vi "Test View No Process Errors Showing and Hiding Panel.vi"(8 "error in (no error)":errorcluster, 11 "UI View Test In":refnum<class "View Test.lvclass">) -> (0 "error out":errorcluster, 3 "UI View Test Out":refnum<class "View Test.lvclass">)   [LabVIEW 2020, in "View Test.lvclass"]
uses:
  View Test.lvclass
  C:/Program Files (x86)/National Instruments/LabVIEW 2020/vi.lib/Astemes/LUnit/Test Case.lvclass
  Mock Error Handler/Mock Error Handler.lvclass
  C:/Git/astemes-triarc-framework/source/Framework/Error Handler Interface/Error Handler Interface.lvclass
  Framework/Process/Process.lvclass/Process.ctl
  Framework/View/View.lvclass/View.ctl
  <vilib>/Astemes/LUnit/Test Case.lvclass/Test Case.ctl
  Framework/Process/Protected/Messaging/Send Message.vi
  Framework/Process/Public/Lifecycle/Get Lifecycle State.vi
  Framework/View/Public/Get View VI Reference.vi
  <vilib>/Utility/error.llb/Clear Errors.vi
  Framework/Broadcast Event Helpers/Execution timer.vi
  Framework/Process/Private/SubVIs/Wait for finish.vi
  Framework/Process/Private/SubVIs/Set Lifecycle State.vi
  <vilib>/Astemes/LUnit/Palette/Pass.vi
  <vilib>/Astemes/LUnit/Palette/Fail.vi
  <vilib>/Astemes/LUnit/Set Assertion Type.vi
  Framework/Process/Private/SubVIs/Handle Debug Data.vi
  Framework/Process/Protected/Messaging/Request Message.vi
  <vilib>/Astemes/LUnit/Add test result.vi
  Framework/Logging/Log Debug.vi
  <vilib>/AdvancedString/1D String Array to Delimited String.vi
  <vilib>/Utility/High Resolution Relative Seconds.vi
  Framework/Process/Private/SubVIs/Enqueue Request Message.vi
  <vilib>/Astemes/LUnit/LUnit Record Assertion Result.vi
  <vilib>/Astemes/LUnit/LUnit Aggregate Assertion Results.vi
  <vilib>/Astemes/LUnit/Method Result/LUnit Merge Status.vi
  <vilib>/Astemes/LUnit/LUnit Concatenate result strings.vi
  Framework/View/View.lvclass
  C:/Git/astemes-triarc-framework/source/Framework/Process/Process.lvclass
  <vilib>/Utility/error.llb/Error Cluster From Error Code.vi
  Framework/Process/Public/Read Name.vi
  Framework/Process/Private/SubVIs/Wait for Response Message.vi
  Framework/Broadcast Event Helpers/Dequeue Broadcast Message.vi
  Framework/Process/Process.lvclass
  View Test.lvclass/View Test.ctl
  <vilib>/Astemes/LUnit/Test Case.lvclass
  C:/Git/astemes-triarc-framework/source/Framework/Base/Base.lvclass
  C:/Git/astemes-triarc-framework/source/Framework/Logging/Logging.lvclass
  C:/Git/astemes-triarc-framework/source/Framework/View/View.lvclass
  Framework/Broadcast Event Helpers/Broadcast Event Helpers.lvlib
  C:/Git/astemes-triarc-framework/source/Framework Test Suite/Process Test/Process Test.lvclass
  C:/Git/astemes-triarc-framework/source/Framework Test Suite/Base Class Test/Base Test.lvclass
  C:/Git/astemes-triarc-framework/source/Framework Test Suite/View Test/View Test.lvclass
  Process Test/Process Test.lvclass
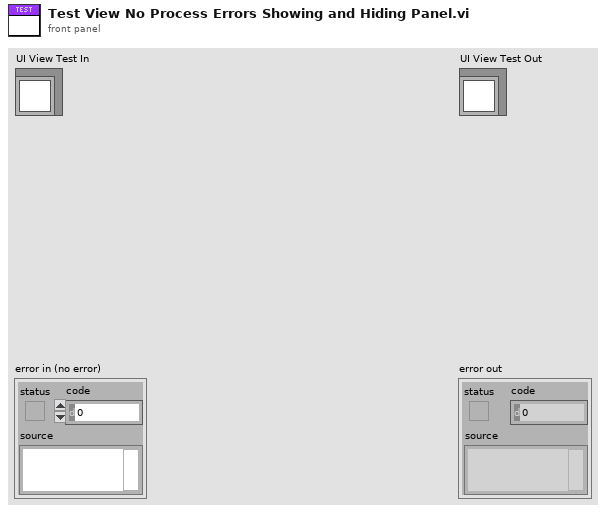
[diagram p1: front panel]
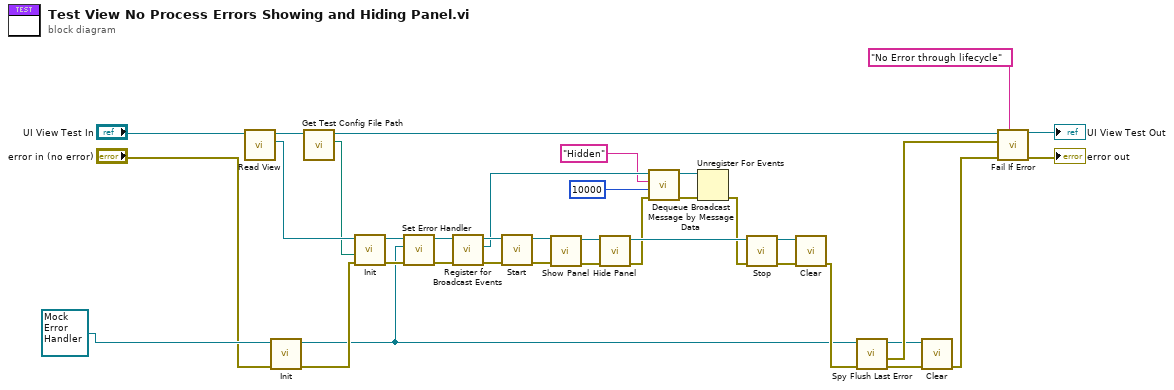
[diagram p0: block diagram]
diagram:
  n1 = call "Read View.vi"("View Test In"="UI View Test In") -> ("View"=w30:refnum<class "View.lvclass">, "View Test Out"=w35:refnum<class "View Test.lvclass">)  [unwired: 8 in, 1 out]
  n2 = call-dynamic "Init.vi"("error in (no error)"="error in (no error)", "Mock Error Handler In"=refnum<class "Mock Error Handler.lvclass"> refnum ("Mock Error Handler.lvclass")) -> ("error out"=w21:errorcluster, "Mock Error Handler Out"=w14:refnum<class "Mock Error Handler.lvclass">)  [unwired: 8 in]
  n3 = call "Get Test Config File Path.vi"("Process Test In"=w35) -> ("Test config path"=w1:path, "Process Test Out"=w2:refnum<class "View Test.lvclass">)  [unwired: 8 in, 1 out]
  n4 = call-dynamic "Init.vi"("error in (no error)"=w21, "Config File Path"=w1, "View In"=w30) -> ("error out"=w24:errorcluster, "View Out"=w32:refnum<class "View.lvclass">)  [unwired: 7 in]
  n5 = call "Set Error Handler.vi"("error in (no error)"=w24, "Error Handler"=w14, "Process In"=w32) -> ("error out"=w23:errorcluster, "Process Out"=w11:refnum<class "View.lvclass">)  [unwired: 7 in]
  n6 = call "Register for Broadcast Events.vi"("error in (no error)"=w23, "Process In"=w11) -> ("error out"=w12:errorcluster, "Event Registration Refnum Out"=w9:refnum<event-registration>, "Process Out"=w10:refnum<class "View.lvclass">)  [unwired: 7 in]
  n7 = call "Start.vi"("error in (no error)"=w12, "Process In"=w10) -> ("error out"=w28:errorcluster, "Process Out"=w29:refnum<class "View.lvclass">)  [unwired: 7 in, 1 out]
  n8 = call "Show Panel.vi"("error in (no error)"=w28, "View In"=w29) -> ("error out"=w16:errorcluster, "View Out"=w17:refnum<class "View.lvclass">)  [unwired: 8 in]
  n9 = call "Hide Panel.vi"("error in (no error)"=w16, "View In"=w17) -> ("error out"=w5:errorcluster, "View Out"=w31:refnum<class "View.lvclass">)  [unwired: 8 in]
  n10 = call "Dequeue Broadcast Message by Message Data.vi"("error in (no error)"=w5, "Timeout (-1)"=10000, "Message Data"="Hidden" ("Message"), "Event Registration Refnum"=w9) -> ("error out"=w4:errorcluster, "Event Registration Refnum Out"=w3:refnum<event-registration>)  [unwired: 3 in, 3 out]
  n11 = Unregister For Events(event registration refnum=w3, error in=w4) -> (error out=w6:errorcluster)
  n12 = call "Stop.vi"("error in (no error)"=w6, "Process In"=w31) -> ("error out"=w26:errorcluster, "Process Out"=w27:refnum<class "View.lvclass">)  [unwired: 7 in, 1 out]
  n13 = call-dynamic "Clear.vi"("error in (no error)"=w26, "View In"=w27) -> ("error out"=w20:errorcluster)  [unwired: 9 in]
  n14 = call "Spy Flush Last Error.vi"("error in (no error)"=w20, "Mock Error Handler In"=w14) -> ("error out"=w18:errorcluster, "Error"=w15:errorcluster, "Mock Error Handler Out"=w13:refnum<class "Mock Error Handler.lvclass">)  [unwired: 7 in]
  n15 = call-dynamic "Clear.vi"("error in (no error)"=w18, "Mock Process In"=w13) -> ("error out"=w19:errorcluster)  [unwired: 9 in]
  n16 = call <vilib>:"Fail If Error.vi"("Description"="No Error through lifecycle", "error in (no error)"=w19, "Assert error"=w15, "LUnit Test Case In"=w2) -> ("error out"=→"error out":errorcluster, "LUnit Test Case Out"=→"UI View Test Out":refnum<class "View Test.lvclass">)  [unwired: 6 in]
